vi "Equal Value Comparison.vi"(6 "verbose? (F)":bool, 8 "error in (no error)":errorcluster, 9 "Actual":variant, 10 "Expected":variant) -> (0 "error out":errorcluster, 2 "Equal Values?":bool, 3 "Verbose output":string)   [LabVIEW 2020, in "Caraya.lvlib" / "Assert.lvclass"]
uses:
  classes/Assert/Assert.lvclass
  classes/Assert/Assert.lvclass/Assert.ctl
  <vilib>/Utility/VariantDataType/VariantType.lvlib
  <userlib>/_OpenG.lib/lvdata/lvdata.llb/openg_variant.lvlib
  <vilib>/Utility/VariantDataType/Type.ctl
  <userlib>/_OpenG.lib/string/string.llb/openg_string.lvlib
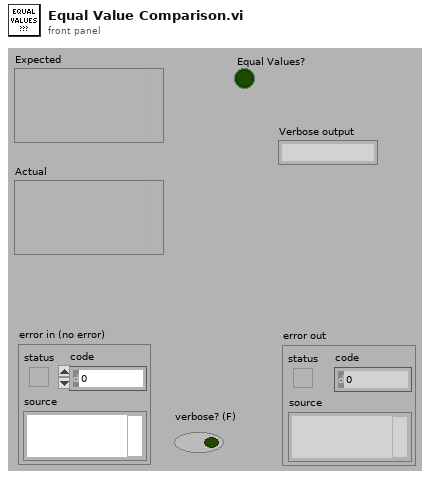
[diagram p1: front panel]
types:
  T1 = typedef "VariantType.lvlib/Type.ctl" = enum8{"Invalid Type", "Void", "I8", "I16", "I32", "I64", "U8", "U16", "U32", "U64", "Single Float", "Double Float", "Extended Float", "Single Complex", "Double Complex", "Extended Complex", "Enum U8", "Enum U16", "Enum U32", "Enum U64", "Single Float With Unit", "Double Float With Unit", "Extended Float With Unit", "Single Complex with Unit", "Double Complex with Unit", "Extended Complex with Unit", "Boolean", "String", "Path", "Picture", "Tag", "Array", "Cluster", "Variant", "LV Variant", "Waveform", "Timestamp", "Digital Waveform", "Digital Data", "ExpressData", "Refnum", "External Data", "VI", "Poly VI", "LabVIEW Class Instance", "Fixed Point"}
  T2 = typedef "openg_variant.lvlib/Physical Units__ogtk.ctl" = cluster{"Base Units":enum16{"radian", "steradian", "second", "meter", "kilogram", "ampere", "kelvin", "mole", "candela"}, "Exponent":i16}
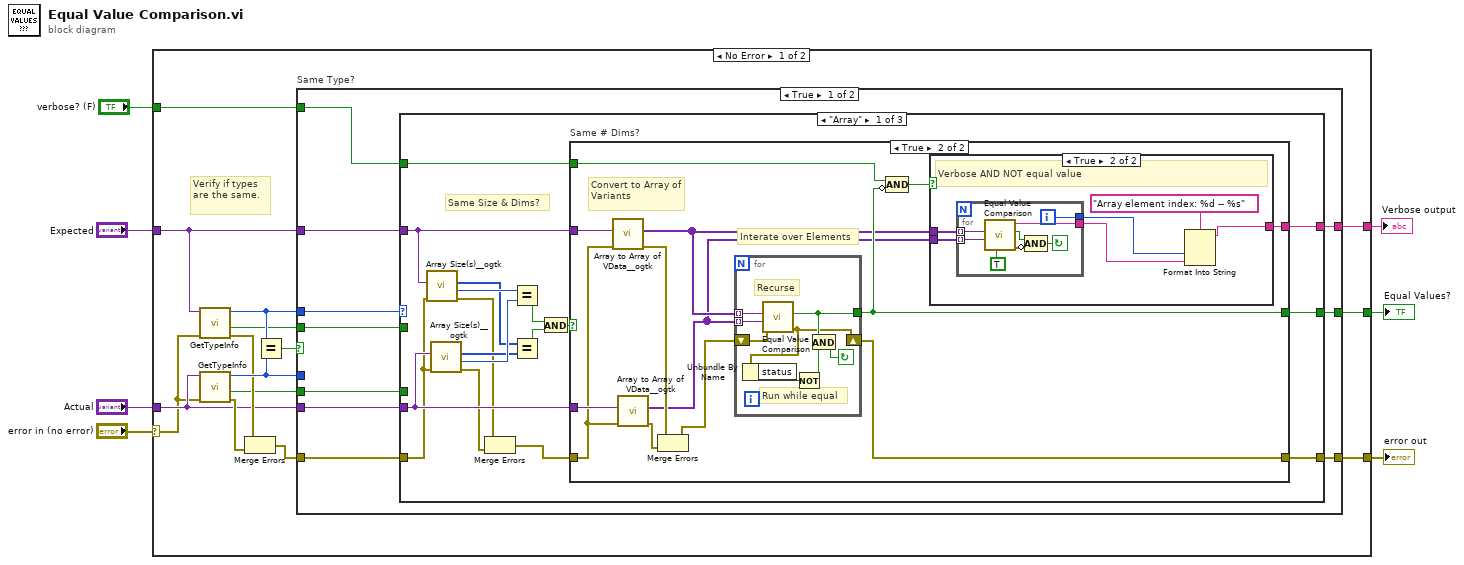
[diagram p0: block diagram]
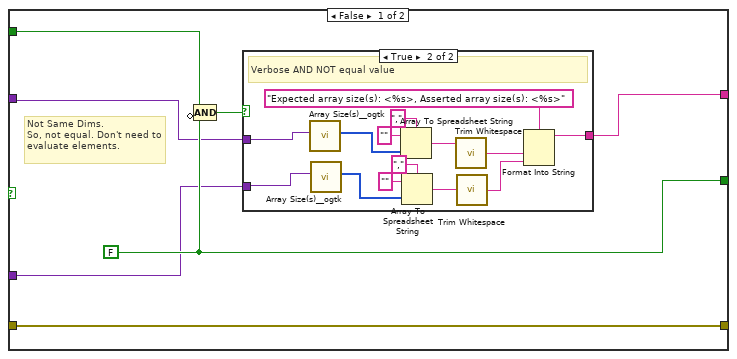
[diagram p2: hidden frame]
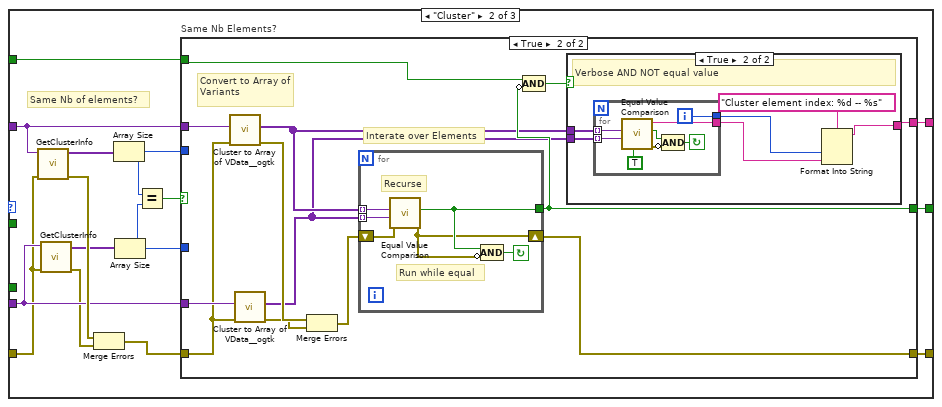
[diagram p5: hidden frame]
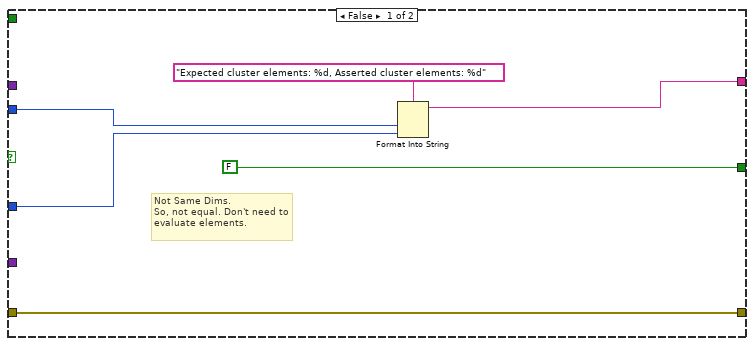
[diagram p6: hidden frame]
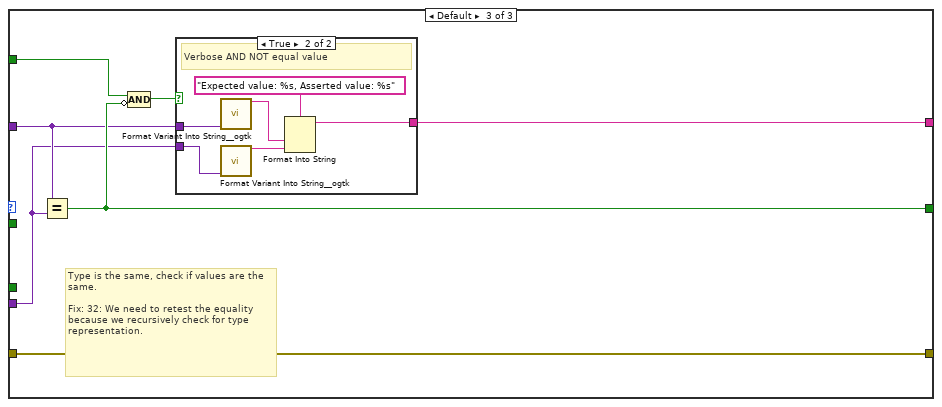
[diagram p8: hidden frame]
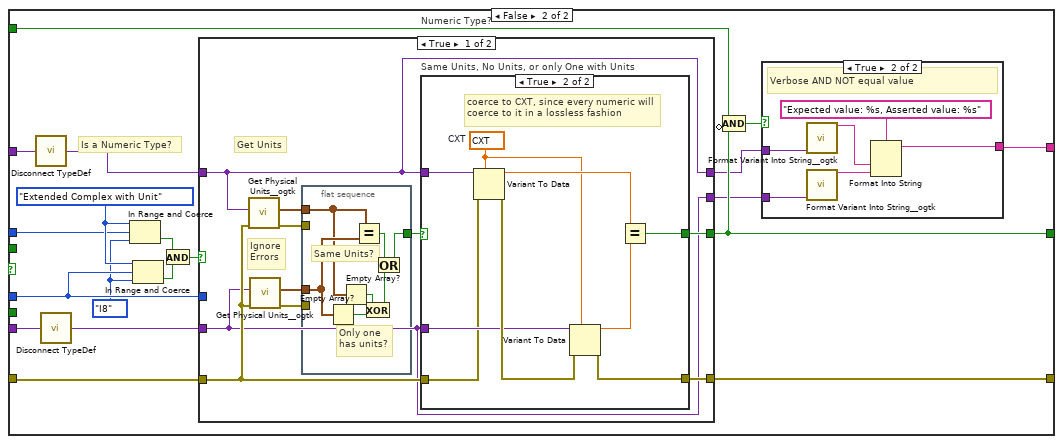
[diagram p10: hidden frame]
diagram:
  n1 = case shown="No Error" "error in (no error)" {
    selector: "error in (no error)" -> [w8 w228]
    tunnel: [w22 _] -> w7
    tunnel: [w21 w228] -> w6
    tunnel: "Actual" -> [w14 _]
    tunnel: "Expected" -> [w13 _]
    tunnel: "verbose? (F)" -> [w10 _]
    tunnel: [w9 _] -> w2
    frame No Error {
      # "Verify if types are the same."
      n2 = call <vilib>:"GetTypeInfo.vi"("error in (no error)"=w8, "Variant"=w13) -> ("error out"=w17:errorcluster, "HasTypedef"=w11:bool, "Type Enum"=w19:T1)  [unwired: 5 in, 2 out]
      n3 = call <vilib>:"GetTypeInfo.vi"("error in (no error)"=w8, "Variant"=w14) -> ("error out"=w16:errorcluster, "HasTypedef"=w12:bool, "Type Enum"=w18:T1)  [unwired: 5 in, 2 out]
      n4 = Merge Errors(w17, w16) -> (w15:errorcluster)
      n5 = Equal?(x=w19, y=w18) -> (x = y?=w20:bool)
      n6 = case "Same Type?" shown="True" w20 {
        tunnel: w13 -> [w30 w182]
        tunnel: w14 -> [w29 w180]
        tunnel: [w32 w177] -> w22
        tunnel: w19 -> [w31 w184]
        tunnel: w18 -> [_ w189]
        tunnel: w15 -> [w28 w191]
        tunnel: [w27 w190] -> w21
        tunnel: w12 -> [w26 _]
        tunnel: w11 -> [w25 _]
        tunnel: w10 -> [w24 w178]
        tunnel: [w23 w173] -> w9
        frame True {
          n7 = case shown="\"Array\"" w31 {
            tunnel: [w35 w120 w165] -> w32
            tunnel: w30 -> [w46 w117 w161]
            tunnel: w29 -> [w47 w114 w160]
            tunnel: w28 -> [w45 w113 w166]
            tunnel: [w49 w119 w166] -> w27
            tunnel: w26 -> [_ _ _]
            tunnel: w25 -> [_ _ _]
            tunnel: w24 -> [w34 w109 w164]
            tunnel: [w33 w106 w162] -> w23
            frame "Array" {
              # "Same Size & Dims?"
              n8 = call <userlib>:"Array Size(s)__ogtk.vi"("error in (no error)"=w45, "Array"=w46) -> ("error out"=w39:errorcluster, "N dims"=w43:u32, "Size(s)"=w41:u32[])  [unwired: 7 in]
              n9 = call <userlib>:"Array Size(s)__ogtk.vi"("error in (no error)"=w45, "Array"=w47) -> ("error out"=w44:errorcluster, "N dims"=w42:u32, "Size(s)"=w40:u32[])  [unwired: 7 in]
              n10 = Merge Errors(w39, w44) -> (w48:errorcluster)
              n11 = Equal?(x=w43, y=w42) -> (x = y?=w37:bool)
              n12 = Equal?(x=w41, y=w40) -> (x = y?=w38:bool)
              n13 = And(x=w37, y=w38) -> (x .and. y?=w36:bool)
              n14 = case "Same # Dims?" shown="True" w36 {
                tunnel: [w53 w74] -> w35
                tunnel: w46 -> [w51 w83]
                tunnel: w47 -> [w50 w82]
                tunnel: [w56 w81] -> w49
                tunnel: w48 -> [w56 w80]
                tunnel: w34 -> [w54 w75]
                tunnel: [w52 w73] -> w33
                frame False {
                  w53 = FALSE ("Equal Values?")
                  # "Not Same Dims.\nSo, not equal. Don't need to evaluate elements."
                  n15 = Compound Arithmetic op=AND(w54, invert w53) -> (w55:bool)
                  n16 = case shown="True" w55 {
                    tunnel: [_ w70] -> w52
                    tunnel: w51 -> [_ w68]
                    tunnel: w50 -> [_ w67]
                    frame False {
                    }
                    frame True {
                      # "Verbose AND NOT equal value"
                      n17 = call <userlib>:"Array Size(s)__ogtk.vi"("Array"=w68) -> ("Size(s)"=w66:u32[])  [unwired: 8 in, 2 out]
                      n18 = call <userlib>:"Array Size(s)__ogtk.vi"("Array"=w67) -> ("Size(s)"=w58:u32[])  [unwired: 8 in, 2 out]
                      n19 = Array To Spreadsheet String(delimiter (Tab)=",", array=w66, 3:"" ("format string")) -> (spreadsheet string=w63:string)
                      n20 = Array To Spreadsheet String(delimiter (Tab)=",", array=w58, 3:"" ("format string")) -> (spreadsheet string=w61:string)
                      n21 = call <vilib>:"Trim Whitespace.vi"("string"=w63) -> ("trimmed string"=w62:string)  [unwired: 1 in]
                      n22 = call <vilib>:"Trim Whitespace.vi"("string"=w61) -> ("trimmed string"=w57:string)  [unwired: 1 in]
                      n23 = Format Into String(format string="Expected array size(s): <%s>, Asserted array size(s): <%s>", w62, w57) -> (resulting string=w70:string)  [unwired: 2 in, 1 out]
                    }
                  }
                }
                frame True {
                  # "Interate over Elements"
                  # "Convert to Array of Variants"
                  n24 = call <userlib>:"Array to Array of VData__ogtk.vi"("error in (no error)"=w80, "MultiD Array"=w83) -> ("error out"=w78:errorcluster, "1D Array of Variants"=w72:variant[])  [unwired: 8 in]
                  n25 = call <userlib>:"Array to Array of VData__ogtk.vi"("error in (no error)"=w80, "MultiD Array"=w82) -> ("error out"=w77:errorcluster, "1D Array of Variants"=w71:variant[])  [unwired: 8 in]
                  n26 = Merge Errors(w78, w77) -> (w79:errorcluster)
                  n27 = for {
                    tunnel: w72 -> [w105] mode=indexing
                    tunnel: w71 -> [w104] mode=indexing
                    tunnel: [w100] -> w74
                    shift-right: [w98] -> w81
                    shift-left: w79 -> [w103]
                    stop <- w99 continue-if-true
                    # "Run while equal"
                    # "Recurse"
                    n28 = call "Equal Value Comparison.vi"("error in (no error)"=w103, "Actual"=w104, "Expected"=w105) -> ("error out"=w98:errorcluster, "Equal Values?"=w100:bool)  [unwired: 6 in, 1 out]
                    n29 = Unbundle By Name(w98) -> ("status"=w101:bool)
                    n30 = Not(x=w101) -> (.not. x?=w102:bool)
                    n31 = And(x=w100, y=w102) -> (x .and. y?=w99:bool)
                  }
                  n32 = Compound Arithmetic op=AND(w75, invert w74) -> (w76:bool)
                  n33 = case shown="True" w76 {
                    tunnel: [_ w86] -> w73
                    tunnel: w72 -> [_ w89]
                    tunnel: w71 -> [_ w88]
                    frame False {
                    }
                    frame True {
                      # "Verbose AND NOT equal value"
                      n34 = for {
                        tunnel: w89 -> [w97] mode=indexing
                        tunnel: w88 -> [w96] mode=indexing
                        tunnel: [w91] -> w85
                        tunnel: [w90] -> w84
                        i -> [w91]
                        stop <- w94 continue-if-true
                        n35 = call "Equal Value Comparison.vi"("verbose? (F)"=TRUE, "Actual"=w96, "Expected"=w97) -> ("error out"=w93:errorcluster, "Equal Values?"=w95:bool, "Verbose output"=w90:string)  [unwired: 6 in]
                        n36 = Compound Arithmetic op=AND(w95, invert w93) -> (w94:bool)
                      }
                      n37 = Format Into String(format string="Array element index: %d -- %s", w85, w84) -> (resulting string=w86:string)  [unwired: 2 in, 1 out]
                    }
                  }
                }
              }
            }
            frame "Cluster" {
              # "Same Nb of elements?"
              n38 = call <vilib>:"GetClusterInfo.vi"("error in (no error)"=w113, "Variant"=w117) -> ("error out"=w115:errorcluster, "Cluster Elements"=w116:variant[])  [unwired: 8 in]
              n39 = call <vilib>:"GetClusterInfo.vi"("error in (no error)"=w113, "Variant"=w114) -> ("error out"=w112:errorcluster, "Cluster Elements"=w110:variant[])  [unwired: 8 in]
              n40 = Merge Errors(w115, w112) -> (w118:errorcluster)
              n41 = Array Size(array=w116) -> (size(s)=w108:i32)
              n42 = Array Size(array=w110) -> (size(s)=w107:i32)
              n43 = Equal?(x=w108, y=w107) -> (x = y?=w111:bool)
              n44 = case "Same Nb Elements?" shown="True" w111 {
                tunnel: [FALSE ("Equal Values?") w130] -> w120
                tunnel: w117 -> [_ w139]
                tunnel: w114 -> [_ w138]
                tunnel: [w125 w137] -> w119
                tunnel: w118 -> [w125 w136]
                tunnel: w109 -> [_ w131]
                tunnel: w108 -> [w124 _]
                tunnel: w107 -> [w123 _]
                tunnel: [w121 w127] -> w106
                frame False {
                  # "Not Same Dims.\nSo, not equal. Don't need to evaluate elements."
                  n45 = Format Into String(format string="Expected cluster elements: %d, Asserted cluster elements: %d", w124, w123) -> (resulting string=w121:string)  [unwired: 2 in, 1 out]
                }
                frame True {
                  # "Interate over Elements"
                  # "Convert to Array of Variants"
                  n46 = call <userlib>:"Cluster to Array of VData__ogtk.vi"("error in (no error)"=w136, "Cluster"=w139) -> ("error out"=w135:errorcluster, "Array of VData"=w129:variant[])  [unwired: 8 in]
                  n47 = call <userlib>:"Cluster to Array of VData__ogtk.vi"("error in (no error)"=w136, "Cluster"=w138) -> ("error out"=w134:errorcluster, "Array of VData"=w128:variant[])  [unwired: 8 in]
                  n48 = Merge Errors(w135, w134) -> (w133:errorcluster)
                  n49 = for {
                    tunnel: w129 -> [w159] mode=indexing
                    tunnel: w128 -> [w158] mode=indexing
                    tunnel: [w156] -> w130
                    shift-right: [w154] -> w137
                    shift-left: w133 -> [w157]
                    stop <- w155 continue-if-true
                    # "Run while equal"
                    # "Recurse"
                    n50 = call "Equal Value Comparison.vi"("error in (no error)"=w157, "Actual"=w158, "Expected"=w159) -> ("error out"=w154:errorcluster, "Equal Values?"=w156:bool)  [unwired: 6 in, 1 out]
                    n51 = Compound Arithmetic op=AND(w156, invert w154) -> (w155:bool)
                  }
                  n52 = Compound Arithmetic op=AND(w131, invert w130) -> (w132:bool)
                  n53 = case shown="True" w132 {
                    tunnel: [_ w142] -> w127
                    tunnel: w129 -> [_ w145]
                    tunnel: w128 -> [_ w144]
                    frame False {
                    }
                    frame True {
                      # "Verbose AND NOT equal value"
                      n54 = for {
                        tunnel: w145 -> [w153] mode=indexing
                        tunnel: w144 -> [w152] mode=indexing
                        tunnel: [w147] -> w141
                        tunnel: [w146] -> w140
                        i -> [w147]
                        stop <- w150 continue-if-true
                        n55 = call "Equal Value Comparison.vi"("verbose? (F)"=TRUE, "Actual"=w152, "Expected"=w153) -> ("error out"=w149:errorcluster, "Equal Values?"=w151:bool, "Verbose output"=w146:string)  [unwired: 6 in]
                        n56 = Compound Arithmetic op=AND(w151, invert w149) -> (w150:bool)
                      }
                      n57 = Format Into String(format string="Cluster element index: %d -- %s", w141, w140) -> (resulting string=w142:string)  [unwired: 2 in, 1 out]
                    }
                  }
                }
              }
            }
            frame Default {
              # "Type is the same, check if values are the same.\n\nFix: 32: We need to retest the equality because we recursively check for type representation."
              n58 = Equal?(x=w161, y=w160) -> (x = y?=w165:bool)
              n59 = Compound Arithmetic op=AND(w164, invert w165) -> (w163:bool)
              n60 = case shown="True" w163 {
                tunnel: [_ w172] -> w162
                tunnel: w161 -> [_ w170]
                tunnel: w160 -> [_ w168]
                frame False {
                }
                frame True {
                  # "Verbose AND NOT equal value"
                  n61 = call <userlib>:"Format Variant Into String__ogtk.vi"("Variant"=w170) -> ("Output String"=w169:string)  [unwired: 13 in, 1 out]
                  n62 = call <userlib>:"Format Variant Into String__ogtk.vi"("Variant"=w168) -> ("Output String"=w167:string)  [unwired: 13 in, 1 out]
                  n63 = Format Into String(format string="Expected value: %s, Asserted value: %s", w169, w167) -> (resulting string=w172:string)  [unwired: 2 in, 1 out]
                }
              }
            }
          }
        }
        frame False {
          w187 = Type."I8" ("Type Enum")
          w188 = Type."Extended Complex with Unit" ("Type Enum")
          # "Is a Numeric Type?"
          n64 = call "Disconnect TypeDef.vi"("Variant"=w182) -> ("Variant Out"=w181:variant)
          n65 = call "Disconnect TypeDef.vi"("Variant"=w180) -> ("Variant Out"=w179:variant)
          n66 = In Range and Coerce(upper limit=w188, x=w184, lower limit=w187) -> (In Range?=w186:bool)  [unwired: 1 out]
          n67 = In Range and Coerce(upper limit=w188, x=w189, lower limit=w187) -> (In Range?=w185:bool)  [unwired: 1 out]
          n68 = And(x=w186, y=w185) -> (x .and. y?=w183:bool)
          n69 = case "Numeric Type?" shown="True" w183 {
            tunnel: w181 -> [w199 w226]
            tunnel: w179 -> [w198 w225]
            tunnel: w189 -> [_ _]
            tunnel: [w207 _] -> w177
            tunnel: w191 -> [w205 w227]
            tunnel: [w206 w227] -> w190
            tunnel: [w199 w226] -> w175
            tunnel: [w198 w225] -> w174
            frame True {
              # "Get Units"
              # "Ignore\nErrors"
              n70 = call <userlib>:"Get Physical Units__ogtk.vi"("error in (no error)"=w205, "Float or Array of Floats"=w199) -> ("error out"=w204:errorcluster, "Physical Units"=w202:T2[])  [unwired: 8 in]
              n71 = call <userlib>:"Get Physical Units__ogtk.vi"("error in (no error)"=w205, "Float or Array of Floats"=w198) -> ("error out"=w203:errorcluster, "Physical Units"=w201:T2[])  [unwired: 8 in]
              n72 = flat-sequence {
                tunnel: w204 -> [_]
                tunnel: w203 -> [_]
                tunnel: w202 -> [w223]
                tunnel: w201 -> [w224]
                tunnel: [w218] -> w200
                frame #0 {
                  # "Same Units?"
                  # "Only one\nhas units?"
                  n73 = Empty Array?(array=w224) -> (empty?=w222:bool)
                  n74 = Empty Array?(array=w223) -> (empty?=w221:bool)
                  n75 = Equal?(x=w223, y=w224) -> (x = y?=w219:bool)
                  n76 = Exclusive Or(1:w222, 2:w221) -> (0:w220:bool)
                  n77 = Or(x=w219, y=w220) -> (x .or. y?=w218:bool)
                }
              }
              n78 = case "Same Units, No Units, or only One with Units" shown="True" w200 {
                tunnel: [_ w217] -> w207
                tunnel: [w208 w216] -> w206
                tunnel: w199 -> [_ w211]
                tunnel: w198 -> [_ w210]
                tunnel: w205 -> [w208 w209]
                frame False {
                  # "Different Units\nCannot have equal value"
                }
                frame True {
                  w212 = cxt 0.0+0.0i  # CXT
                  # "coerce to CXT, since every numeric will coerce to it in a lossless fashion"
                  n79 = Variant To Data(error in=w209, type=w212, Variant=w211) -> (data=w215:cxt, error out=w213:errorcluster)
                  n80 = Variant To Data(error in=w213, type=w212, Variant=w210) -> (data=w214:cxt, error out=w216:errorcluster)
                  n81 = Equal?(x=w215, y=w214) -> (x = y?=w217:bool)
                }
              }
            }
            frame False {
              # "All non-integer representations must be of same type to potentially assert True,"
            }
          }
          n82 = Compound Arithmetic op=AND(w178, invert w177) -> (w176:bool)
          n83 = case shown="True" w176 {
            tunnel: [_ w197] -> w173
            tunnel: w175 -> [_ w195]
            tunnel: w174 -> [_ w193]
            frame False {
            }
            frame True {
              # "Verbose AND NOT equal value"
              n84 = call <userlib>:"Format Variant Into String__ogtk.vi"("Variant"=w195) -> ("Output String"=w194:string)  [unwired: 13 in, 1 out]
              n85 = call <userlib>:"Format Variant Into String__ogtk.vi"("Variant"=w193) -> ("Output String"=w192:string)  [unwired: 13 in, 1 out]
              n86 = Format Into String(format string="Expected value: %s, Asserted value: %s", w194, w192) -> (resulting string=w197:string)  [unwired: 2 in, 1 out]
            }
          }
        }
      }
    }
    frame Error {
    }
  }
  "Equal Values?" <- w7
  "error out" <- w6
  "Verbose output" <- w2
